vi "Next_Core.vi"(8 "error in (no error)":errorcluster, 10 "PGJDPResult in":refnum<class "Result.lvclass">, 11 "SqlMapper in":refnum<class "SqlMapper.lvclass">) -> (0 "error out":errorcluster, 1 "Found":bool, 2 "Row as Variant":variant, 3 "SqlMapper out":refnum<class "SqlMapper.lvclass">)   [LabVIEW 2020, in "ORM_pgsql_jdp.lvlib" / "Result.lvclass"]
uses:
  Result.lvclass
  <vilib>/Viviota/shared/ORM.lvlibp/SqlMapper/SqlMapper.lvclass
  Result.lvclass/Result.ctl
  <vilib>/JDP Science/PostgreSQL Library/Result/PQ Result.lvclass/PQ Result.ctl
  <vilib>/JDP Science/PostgreSQL Library/Result/Write Next Column.vi
  <vilib>/JDP Science/PostgreSQL Library/Result/Get Variant.vi
  <vilib>/JDP Science/PostgreSQL Library/Result/Number of Columns.vi
  <vilib>/JDP Science/PostgreSQL Library/Result/Write Next Row.vi
  <vilib>/JDP Science/PostgreSQL Library/Result/Get Column String.vi
  <vilib>/JDP Science/PostgreSQL Library/Result/subVIs/PQ DVR Error.vi
  <vilib>/JDP Science/PostgreSQL Library/Result/Read Next Row.vi
  <vilib>/JDP Science/PostgreSQL Library/Result/Get Column Headers.vi
  <vilib>/JDP Science/PostgreSQL Library/Result/Get IsNull.vi
  <vilib>/JDP Science/PostgreSQL Library/Result/Get Type.vi
  <vilib>/JDP Science/PostgreSQL Library/Result/Get ByteA.vi
  <vilib>/Utility/error.llb/Error Cluster From Error Code.vi
  <vilib>/JDP Science/PostgreSQL Library/Result/Get Column I64.vi
  <vilib>/JDP Science/PostgreSQL Library/Result/Get Column DBL.vi
  <vilib>/JDP Science/PostgreSQL Library/Result/Get Column Boolean.vi
  <vilib>/JDP Science/PostgreSQL Library/Result/Get Column Timestamp.vi
  <vilib>/JDP Science/PostgreSQL Library/Result/Get Column I64[].vi
  <vilib>/JDP Science/PostgreSQL Library/Result/Get Column DBL[].vi
  <vilib>/JDP Science/PostgreSQL Library/Result/Get Column SGL[].vi
  <vilib>/JDP Science/PostgreSQL Library/Result/Get String[].vi
  <vilib>/JDP Science/PostgreSQL Library/Result/PQ Result.lvclass
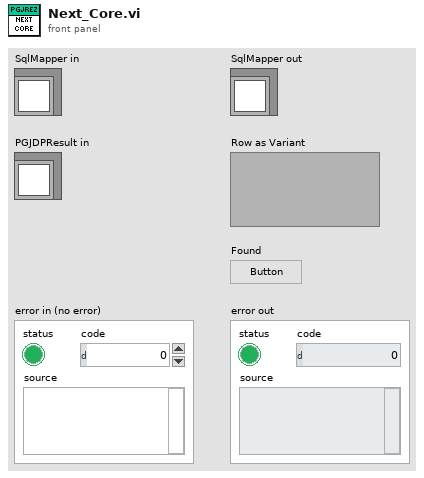
[diagram p1: front panel]
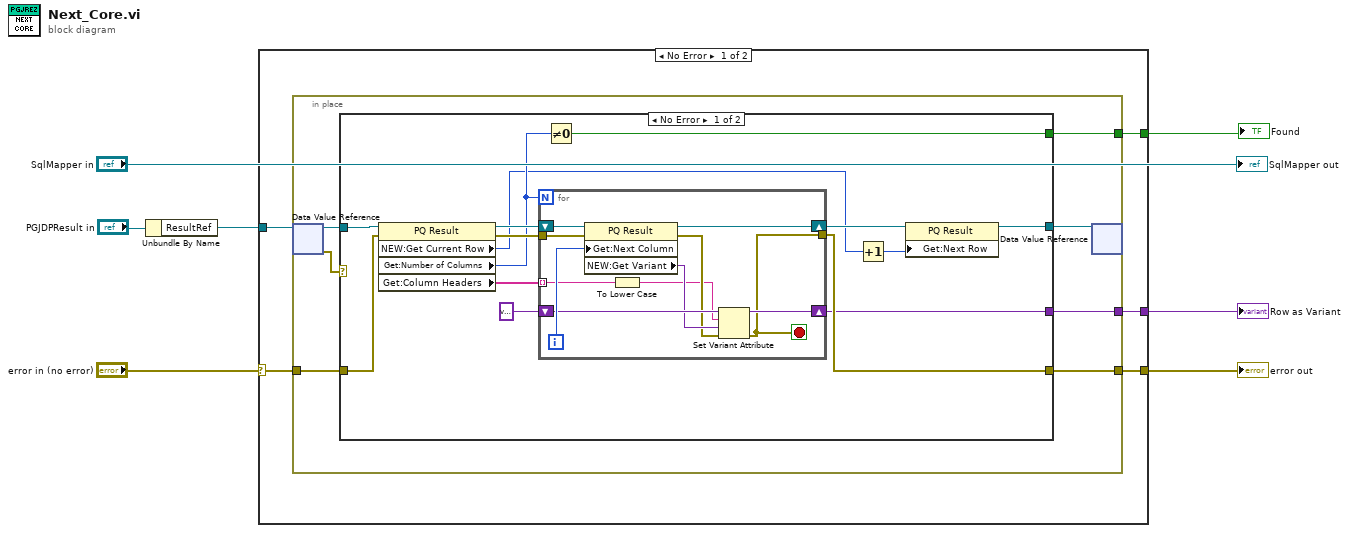
[diagram p0: block diagram]
diagram:
  n1 = Unbundle By Name("PGJDPResult in") -> ("ResultRef"=w2:refnum<data-value>)
  n2 = case shown="No Error" "error in (no error)" {
    selector: "error in (no error)" -> [w12 w47]
    tunnel: [w11 w47] -> w4
    tunnel: [w10 _] -> w3
    tunnel: w2 -> [w9 _]
    tunnel: [w8 _] -> w1
    frame No Error {
      n3 = in-place {
        in-place-border: w12 -> [w19]
        in-place-border: [w18] -> w11
        in-place-border: [w17] -> w10
        in-place-border: [w14] -> w8
        n4 = in-place-dvr #1(w9) -> (w16:refnum<class "PQ Result.lvclass">, w13:errorcluster)
        n5 = case shown="No Error" w13 {
          selector: w13 -> [_ w46]
          tunnel: w19 -> [w29 _]
          tunnel: [w28 w46] -> w18
          tunnel: [w27 _] -> w17
          tunnel: w16 -> [w22 w45]
          tunnel: [w21 w45] -> w15
          tunnel: [w20 _] -> w14
          frame No Error {
            n6 = property class="PQ Result"(reference=w22, error in=w29) -> (reference out=w33:refnum<class "PQ Result.lvclass">, error out=w30:errorcluster, "NEW:Get Current Row"=w24:i32, "Get:Number of Columns"=w26:i32, "Get:Column Headers"=w32:string[])
            n7 = for {
              N: w26 -> [_]
              tunnel: w32 -> [w39] mode=indexing
              shift-right: [w41] -> w27
              shift-left: variant -> [w42]
              tunnel: w30 -> [w37]
              tunnel: [w36] -> w28
              shift-right: [w34] -> w25
              shift-left: w33 -> [w44]
              i -> [w43]
              stop <- w36 stop-if-true
              n8 = property class="PQ Result"(reference=w44, error in=w37, "Get:Next Column"=w43) -> (reference out=w34:refnum<class "PQ Result.lvclass">, error out=w38:errorcluster, "NEW:Get Variant"=w40:variant)
              n9 = To Lower Case(string=w39) -> (all lower case string=w35:string)
              n10 = Set Variant Attribute(Variant=w42, name=w35, value=w40, error in=w38) -> (Variant out=w41:variant, error out=w36:errorcluster)  [unwired: 1 out]
            }
            n11 = Not Equal To 0?(x=w26) -> (x != 0?=w20:bool)
            n12 = Increment(x=w24) -> (x+1=w23:i32)
            n13 = property class="PQ Result"(reference=w25, "Get:Next Row"=w23) -> (reference out=w21:refnum<class "PQ Result.lvclass">)  [unwired: 1 in, 1 out]
          }
          frame Error {
          }
        }
        n14 = in-place-dvr #1(w15) -> ()  [unwired: 2 out]
      }
    }
    frame Error {
    }
  }
  "error out" <- w4
  "Row as Variant" <- w3
  "Found" <- w1
  "SqlMapper out" <- "SqlMapper in"
